vi "Make Command Wrappers.vi"(6 "Search String":string=" Immediate.vi", 8 "error in (no error)":errorcluster, 9 "Imm Cmds":string[](array[string]), 10 "VI Refs":refnum<vi>[](array[refnum]), 11 "Subsystem Name":string) -> (0 "error out":errorcluster)   [LabVIEW 2025]
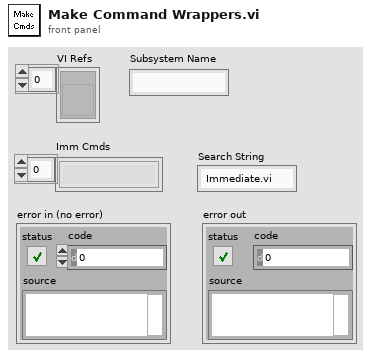
[diagram p1: front panel]
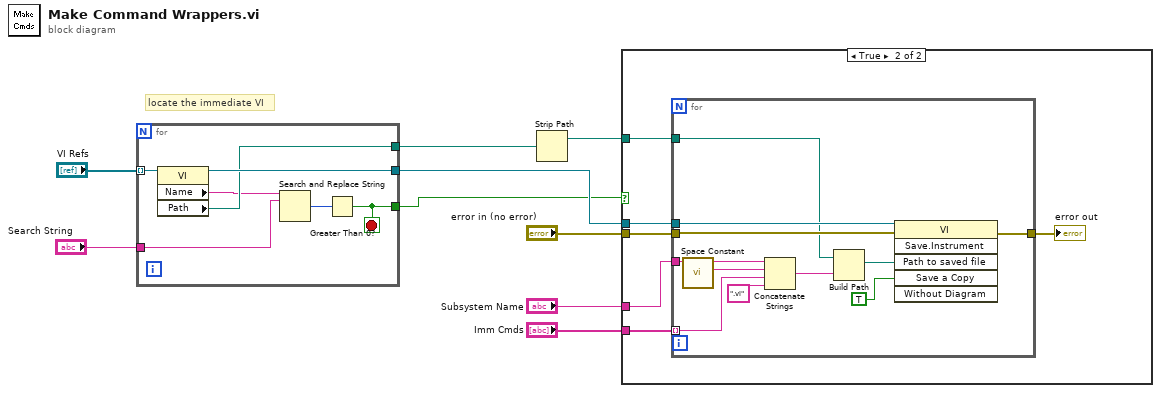
[diagram p0: block diagram]
diagram:
  # "locate the immediate VI"
  n1 = for {
    tunnel: "VI Refs" -> [w15] mode=indexing
    tunnel: [w11] -> w2
    tunnel: [w14] -> w6
    tunnel: [w13] -> w5
    tunnel: "Search String" -> [w10]
    stop <- w11 stop-if-true
    n2 = property class="VI"(reference=w15) -> (reference out=w14:refnum<vi>, "Name"=w12:string, "Path"=w13:path)  [unwired: 1 in, 1 out]
    n3 = Search and Replace String(input string=w12, search string=w10) -> (number of replacements=w16:i32)  [unwired: 6 in, 3 out]
    n4 = Greater Than 0?(x=w16) -> (x > 0?=w11:bool)
  }
  n5 = Strip Path(path=w5) -> (stripped path=w4:path)  [unwired: 1 out]
  n6 = case shown="True" w2 {
    tunnel: "error in (no error)" -> [_ w21]
    tunnel: "Imm Cmds" -> [_ w20]
    tunnel: w6 -> [_ w19]
    tunnel: w4 -> [_ w18]
    tunnel: "Subsystem Name" -> [_ w17]
    frame False {
    }
    frame True {
      n7 = for {
        tunnel: w19 -> [w32]
        tunnel: w21 -> [w31]
        tunnel: [w28] -> w22
        tunnel: w20 -> [w27] mode=indexing
        tunnel: w18 -> [w30]
        tunnel: w17 -> [w26]
        n8 = call <vilib>:"Space Constant.vi"() -> ("String"=w25:string)
        n9 = Concatenate Strings(w26, w25, w27, ".vi") -> (w24:string)
        n10 = Build Path(base path=w30, name or relative path=w24) -> (appended path=w33:path)
        n11 = invoke class="VI" method="Save.Instrument"(reference=w32, error in=w31, "Path to saved file"=w33, "Save a Copy"=TRUE) -> (error out=w28:errorcluster)  [unwired: 2 in, 5 out]
      }
      "error out" <- w22
    }
  }
